vi "KeyPressLUT.vi"(7 "Keyboard No Op":bool, 8 "error in (no error)":errorcluster, 9 "Keyboard Key Pressed":T2(ring), 10 "Sample Number":u32, 11 "LUT Selector":T3) -> (0 "error out":errorcluster, 3 "KeyboardKeysPressed":T1(array[ring]))   [LabVIEW 2026, in "Core.lvlib"]
uses:
  modules/coordinator/src/Libraries/Core/Core.lvlib
  modules/coordinator/src/Libraries/KeyboardLUTSelector.ctl
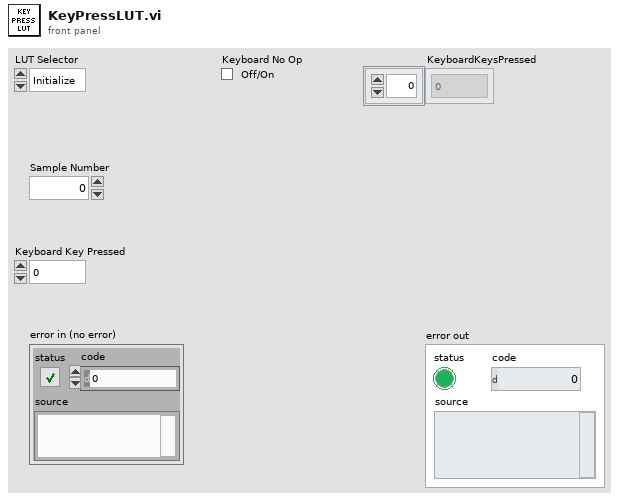
[diagram p1: front panel]
types:
  T1 = enum16{"0", "1", "2", "3", "4", "5", "6", "7", "8", "9", "A", "B", "C", "D", "E", "F", "G", "H", "I", "J", "K", "L", "M", "N", "O", "P", "Q", "R", "S", "T", "U", "V", "W", "X", "Y", "Z", "F1", "F2", "F3", "F4", "F5", "F6", "F7", "F8", "F9", "F10", "F11", "F12", "F13", "F14", "F15", "ADD", "BACK", "BACKSLASH", "CAPITAL", "COMMA", "DECIMAL", "DELETE", "DIVIDE", "DOWN", "END", "EQUALS", "ESCAPE", "GRAVE (`)", "HOME", "INSERT", "LBRACKET", "LCONTROL", "LEFT", "L ALT", "LSHIFT", "LWIN", "MINUS", "MULTIPLY", "NEXT", "NUMLOCK", "NUMPAD_0", "NUMPAD_1", "NUMPAD_2", "NUMPAD_3", "NUMPAD_4", "NUMPAD_5", "NUMPAD_6", "NUMPAD_7", "NUMPAD_8", "NUMPAD_9", "PAUSE", "PERIOD", "PRIOR (PG UP)", "RBRACKET", "RCONTROL", "RETURN", "RIGHT", "R ALT", "RSHIFT", "RWIN", "SCROLL", "SEMICOLON", "SLASH", "SPACE", "SUBTRACT", "TAB", "UP", "ENTER (num pad)", "' (quote)"}[]
  T2 = enum16{"0", "1", "2", "3", "4", "5", "6", "7", "8", "9", "A", "B", "C", "D", "E", "F", "G", "H", "I", "J", "K", "L", "M", "N", "O", "P", "Q", "R", "S", "T", "U", "V", "W", "X", "Y", "Z", "F1", "F2", "F3", "F4", "F5", "F6", "F7", "F8", "F9", "F10", "F11", "F12", "F13", "F14", "F15", "ADD", "BACK", "BACKSLASH", "CAPITAL", "COMMA", "DECIMAL", "DELETE", "DIVIDE", "DOWN", "END", "EQUALS", "ESCAPE", "GRAVE (`)", "HOME", "INSERT", "LBRACKET", "LCONTROL", "LEFT", "L ALT", "LSHIFT", "LWIN", "MINUS", "MULTIPLY", "NEXT", "NUMLOCK", "NUMPAD_0", "NUMPAD_1", "NUMPAD_2", "NUMPAD_3", "NUMPAD_4", "NUMPAD_5", "NUMPAD_6", "NUMPAD_7", "NUMPAD_8", "NUMPAD_9", "PAUSE", "PERIOD", "PRIOR (PG UP)", "RBRACKET", "RCONTROL", "RETURN", "RIGHT", "R ALT", "RSHIFT", "RWIN", "SCROLL", "SEMICOLON", "SLASH", "SPACE", "SUBTRACT", "TAB", "UP", "ENTER (num pad)", "' (quote)"}
  T3 = typedef "Core.lvlib/KeyboardLUTSelector.ctl" = enum16{"Initialize", "Get Keyboards Keys Pressed at Sample Number", "Assign Keyboard Key Press to Sample Number"}
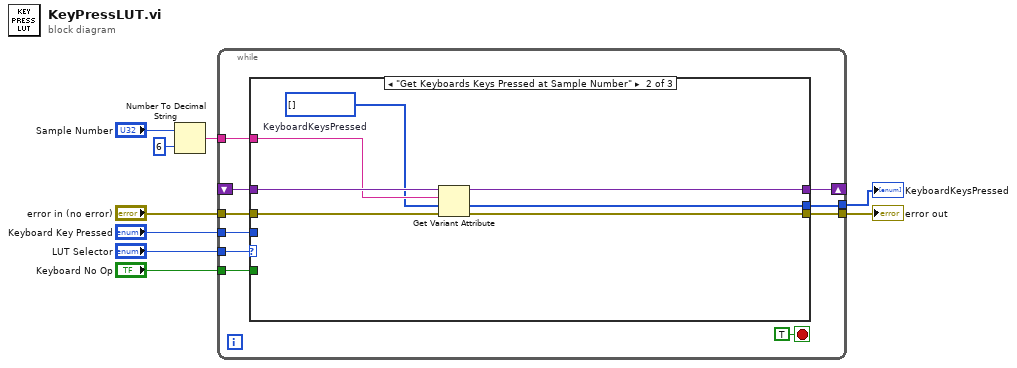
[diagram p0: block diagram]
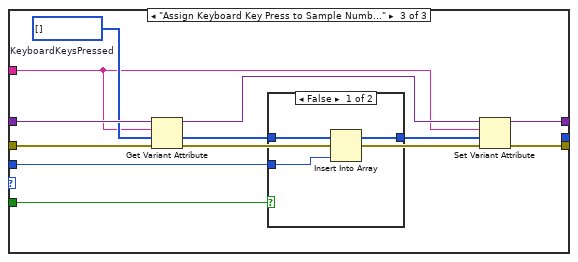
[diagram p3: hidden frame]
diagram:
  n1 = Number To Decimal String(number="Sample Number", width (-)=i16 6) -> (decimal integer string=w3:string)
  n2 = while {
    tunnel: "LUT Selector" -> [w18]
    shift-right: [w17] -> _
    shift-left: _ -> [w16]
    tunnel: w3 -> [w15]
    tunnel: [w14] -> w8
    tunnel: "Keyboard Key Pressed" -> [w13]
    tunnel: [w11] -> w6
    tunnel: "Keyboard No Op" -> [w12]
    tunnel: "error in (no error)" -> [w10]
    stop <- TRUE stop-if-true
    n3 = case shown="\"Get Keyboards Keys Pressed at Sample Number\"" w18 {
      tunnel: [variant w27 w35] -> w17
      tunnel: w16 -> [_ w28 w40]
      tunnel: w15 -> [_ w25 w32]
      tunnel: [w20 w26 w33] -> w14
      tunnel: w13 -> [_ _ w34]
      tunnel: w12 -> [_ _ w30]
      tunnel: [_ w23 _] -> w11
      tunnel: w10 -> [w20 w22 w29]
      frame "Initialize", Default {
      }
      frame "Get Keyboards Keys Pressed at Sample Number" {
        w24 = T1 [] items=["0", "1", "2", "3", "4", "5", "6", "7", "8", "9", "A", "B", "C", "D", "E", "F", "G", "H", "I", "J", "K", "L", "M", "N", "O", "P", "Q", "R", "S", "T", "U", "V", "W", "X", "Y", "Z", "F1", "F2", "F3", "F4", "F5", "F6", "F7", "F8", "F9", "F10", "F11", "F12", "F13", "F14", "F15", "ADD", "BACK", "BACKSLASH", "CAPITAL", "COMMA", "DECIMAL", "DELETE", "DIVIDE", "DOWN", "END", "EQUALS", "ESCAPE", "GRAVE (`)", "HOME", "INSERT", "LBRACKET", "LCONTROL", "LEFT", "L ALT", "LSHIFT", "LWIN", "MINUS", "MULTIPLY", "NEXT", "NUMLOCK", "NUMPAD_0", "NUMPAD_1", "NUMPAD_2", "NUMPAD_3", "NUMPAD_4", "NUMPAD_5", "NUMPAD_6", "NUMPAD_7", "NUMPAD_8", "NUMPAD_9", "PAUSE", "PERIOD", "PRIOR (PG UP)", "RBRACKET", "RCONTROL", "RETURN", "RIGHT", "R ALT", "RSHIFT", "RWIN", "SCROLL", "SEMICOLON", "SLASH", "SPACE", "SUBTRACT", "TAB", "UP", "ENTER (num pad)", "' (quote)"]  # KeyboardKeysPressed
        n4 = Get Variant Attribute(Variant=w28, name=w25, default value (empty Variant)=w24, error in=w22) -> (duplicate Variant=w27:variant, value=w23:T1, error out=w26:errorcluster)  [unwired: 1 out]
      }
      frame "Assign Keyboard Key Press to Sample Number" {
        w37 = T1 [] items=["0", "1", "2", "3", "4", "5", "6", "7", "8", "9", "A", "B", "C", "D", "E", "F", "G", "H", "I", "J", "K", "L", "M", "N", "O", "P", "Q", "R", "S", "T", "U", "V", "W", "X", "Y", "Z", "F1", "F2", "F3", "F4", "F5", "F6", "F7", "F8", "F9", "F10", "F11", "F12", "F13", "F14", "F15", "ADD", "BACK", "BACKSLASH", "CAPITAL", "COMMA", "DECIMAL", "DELETE", "DIVIDE", "DOWN", "END", "EQUALS", "ESCAPE", "GRAVE (`)", "HOME", "INSERT", "LBRACKET", "LCONTROL", "LEFT", "L ALT", "LSHIFT", "LWIN", "MINUS", "MULTIPLY", "NEXT", "NUMLOCK", "NUMPAD_0", "NUMPAD_1", "NUMPAD_2", "NUMPAD_3", "NUMPAD_4", "NUMPAD_5", "NUMPAD_6", "NUMPAD_7", "NUMPAD_8", "NUMPAD_9", "PAUSE", "PERIOD", "PRIOR (PG UP)", "RBRACKET", "RCONTROL", "RETURN", "RIGHT", "R ALT", "RSHIFT", "RWIN", "SCROLL", "SEMICOLON", "SLASH", "SPACE", "SUBTRACT", "TAB", "UP", "ENTER (num pad)", "' (quote)"]  # KeyboardKeysPressed
        n5 = Get Variant Attribute(Variant=w40, name=w32, default value (empty Variant)=w37, error in=w29) -> (duplicate Variant=w39:variant, value=w36:T1, error out=w38:errorcluster)  [unwired: 1 out]
        n6 = case shown="False" w30 {
          tunnel: w36 -> [w43 w44]
          tunnel: w34 -> [w42 _]
          tunnel: [w41 w44] -> w31
          frame False {
            n7 = Insert Into Array(array=w43, new element=w42) -> (w41:T1)  [unwired: 1 in]
          }
          frame True {
          }
        }
        n8 = Set Variant Attribute(Variant=w39, name=w32, value=w31, error in=w38) -> (Variant out=w35:variant, error out=w33:errorcluster)  [unwired: 1 out]
      }
    }
  }
  "error out" <- w8
  "KeyboardKeysPressed" <- w6
